vi "Repeat.vi"(11 "CSM Name":string="Repeat") -> ()   [LabVIEW 2026, in "UI-步进.lvlib" / "Repeat.lvlib"]
uses:
  Repeat.lvlib
  Supports/Repeat Steps.ctl
  Supports/Repeating States.ctl
  <userlib>/_NEVSTOP/Communicable State Machine(CSM)/_Polymophic/CSM - Filter Duplicated Lines.vi
  816fba94-53db-458f-9fde-c2796c7a1569.vi
  ea879a80-eb10-4c3f-a93b-bc01ba185342.vi
  ba2d9a0e-10df-4741-bda9-2194bb22ae09.vi
  84c4a0cb-90b1-43d3-96e0-8d2f37924e74.vi
  ccb58757-6b9e-4b1a-98c8-8aa3e3073145.vi
  b9097fe4-5901-4bf7-874c-569f3441d03a.vi
  be3ae19b-8a37-463e-a95d-eee2ed27764c.vi
  05157bae-8af7-4530-8df5-f99514427171.vi
  <userlib>/_NEVSTOP/Communicable State Machine(CSM)/_Polymophic/CSM - Replace Marks in Messages.vi
  2c826c22-9728-4daa-abad-67d06329c265.vi
  1395e5c4-d7de-483e-aee6-084de6ff1113.vi
  <userlib>/_NEVSTOP/Communicable State Machine(CSM)/AdvanceAPI/CSM - Compact Multiple States.vi
  <userlib>/_NEVSTOP/Communicable State Machine(CSM)/AdvanceAPI/CSM - Break Down Multiple States String.vi
  <userlib>/_NEVSTOP/Communicable State Machine(CSM)/_Shared/Remove Comments from Single-line.vi
  <userlib>/_NEVSTOP/Communicable State Machine(CSM)/_Shared/Split Single-line Message.vi
  <userlib>/_NEVSTOP/Communicable State Machine(CSM)/_Shared/Trim Single-line Text.vi
  <userlib>/_NEVSTOP/Communicable State Machine(CSM)/AdvanceAPI/CSM - Revert Arguments-Safe String.vi
  <userlib>/_NEVSTOP/Communicable State Machine(CSM)/AdvanceAPI/CSM - Make String Arguments Safe.vi
  <userlib>/_NEVSTOP/Communicable State Machine(CSM)/AdvanceAPI/CSM - Keywords.vi
  <userlib>/_NEVSTOP/Communicable State Machine(CSM)/AdvanceAPI/CSM - Get Module Attribute.vi
  <userlib>/_NEVSTOP/Communicable State Machine(CSM)/addons/API-String-Arugments-Support/_Support/Convert API String Arguments to Data(variant).vi
  <userlib>/_NEVSTOP/Communicable State Machine(CSM)/addons/API-String-Arugments-Support/_Support/Data To API String Arguments.vi
  <userlib>/_NEVSTOP/Communicable State Machine(CSM)/Communicable State Machine.lvlib
  <userlib>/_NEVSTOP/Communicable State Machine(CSM)/addons/Loop-Support/CSM Loop Support.lvlib
  <userlib>/_NEVSTOP/Communicable State Machine(CSM)/addons/INI-Static-Variable-Support/INI-Static-Variable-Support.lvlib
panel:
  in  "运行次数":dbl=inf format="%#.0f"
  out "当前次数":i32
  in  "循环开始":bool
  in  "电机步骤":T1=[{"行程"=25, "周期"=600, "进度"=0.0, "光谱测量拿起"=FALSE, "运行方向"=FALSE}, {"行程"=25, "周期"=600, "进度"=0.0, "光谱测量拿起"=FALSE, "运行方向"=FALSE}, {"行程"=25, "周期"=600, "进度"=0.0, "光谱测量拿起"=FALSE, "运行方向"=FALSE}, {"行程"=25, "周期"=600, "进度"=0.0, "光谱测量拿起"=FALSE, "运行方向"=FALSE}] {"进度" scale=0.0..1.0}
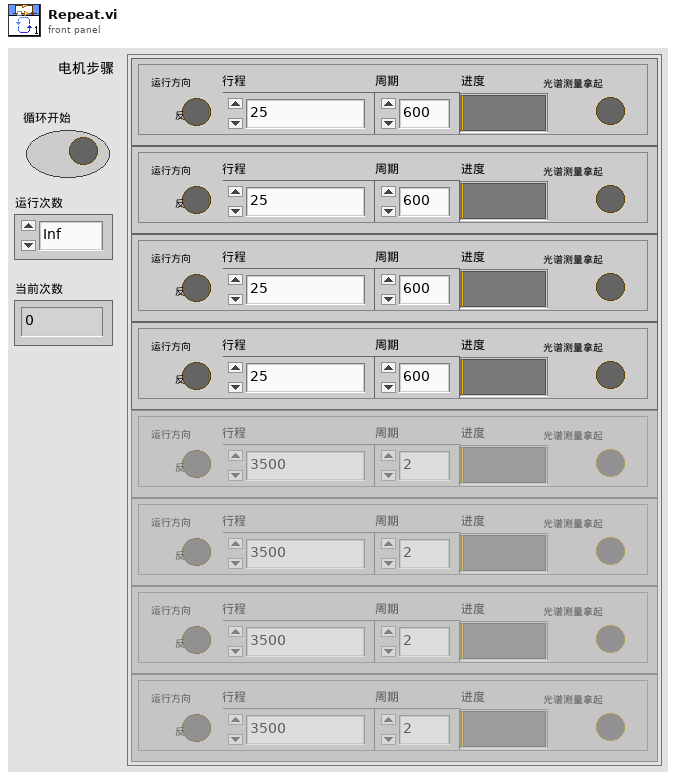
[diagram p1: front panel]
types:
  T1 = typedef "UI-步进.lvlib/Repeat Steps.ctl" = cluster{"行程":i32, "周期":i32, "进度":dbl, "光谱测量拿起":bool, "运行方向":bool}[]
  T2 = enum32{"Invalid", "Standard", "Closed", "Hidden", "Minimized", "Maximized"}
  T3 = enum32{"invalid app kind", "Development System", "Run Time System", "Student Edition", "Embedded LabVIEW", "Evaluation", "Custom"}
  T4 = typedef "UI-步进.lvlib/Repeat.lvlib/Repeating States.ctl" = enum16{"Idle", "Repeating", "Error"}
  T5 = typedef "Communicable State Machine.lvlib/_CSM_Response Source Message.ctl" = cluster{"‘State":string, "’Arguments":string, "’Error":errorcluster}
  T6 = cluster{"Current VI Reference":refnum<vi>, "Close Panel on Exit?":bool}
  T7 = cluster{"Core":cluster{"Current VI Reference":refnum<vi>, "Close Panel on Exit?":bool}, "State":T4, "Repeat":cluster{"电机步骤开始时间":timestamp, "电机步骤索引":i32[], "下一步？":bool, "步骤开始周期":i32}, "CSM Name":string, "INI Path":path}
  T8 = cluster{"电机步骤开始时间":timestamp, "电机步骤索引":i32[], "下一步？":bool, "步骤开始周期":i32}
  T9 = cluster{"行程":i32, "周期":i32, "进度":dbl, "光谱测量拿起":bool, "运行方向":bool}
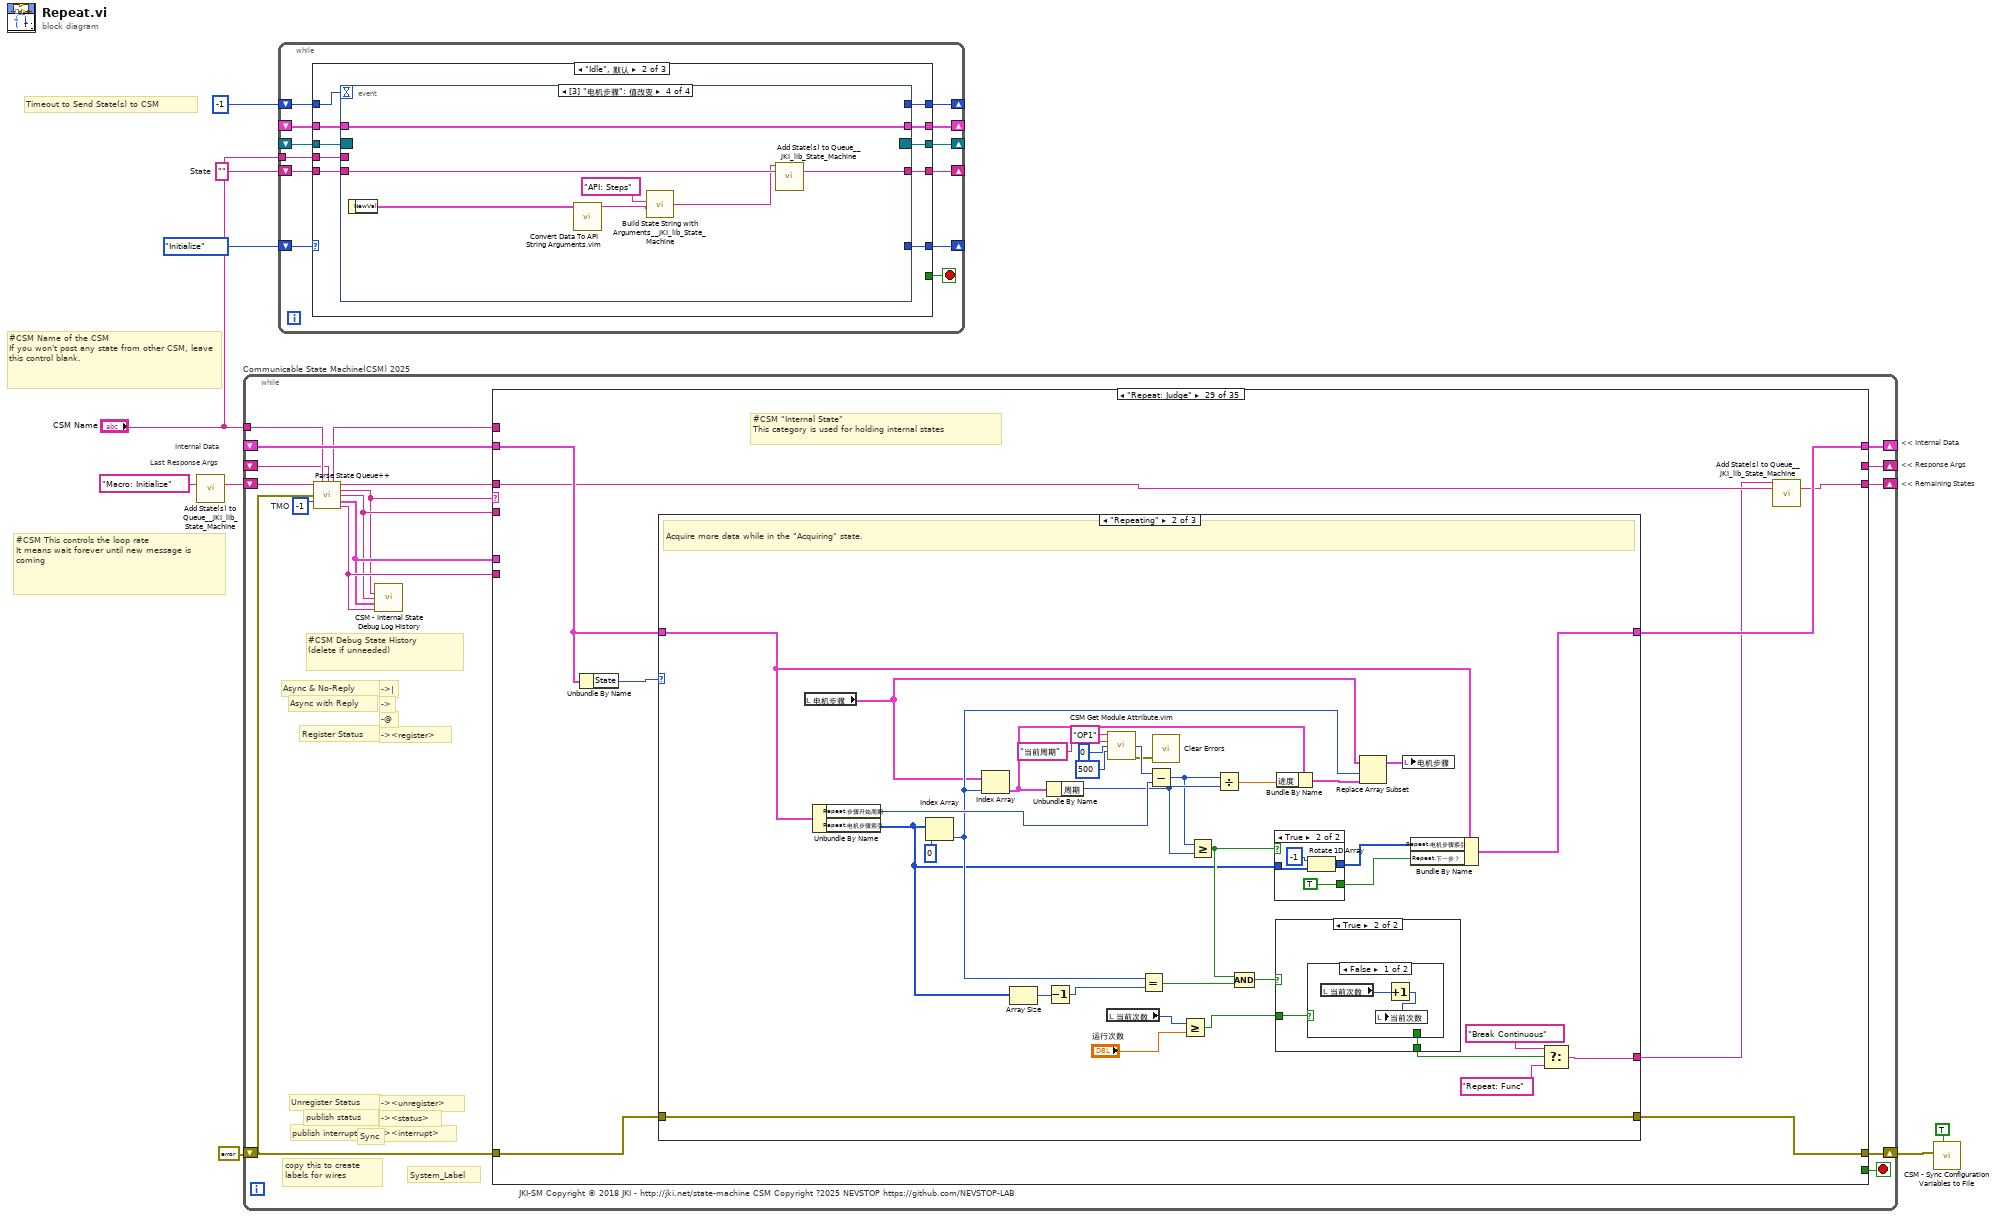
[diagram p0: block diagram]
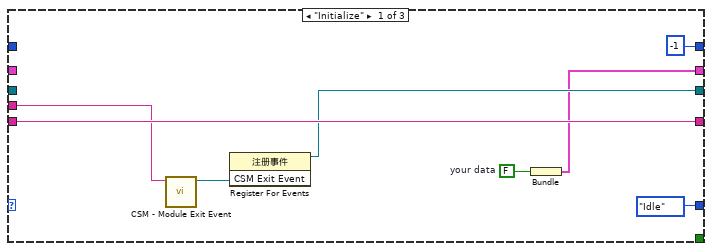
[diagram p2: hidden frame]
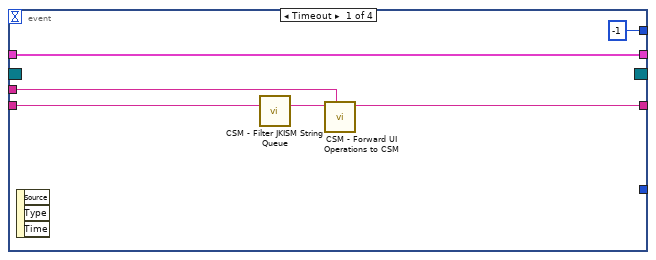
[diagram p3: hidden frame]
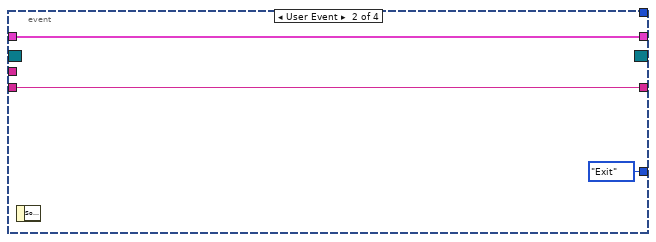
[diagram p4: hidden frame]
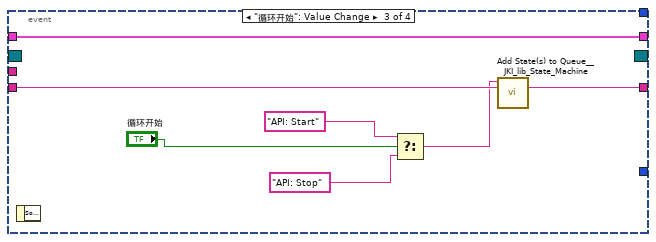
[diagram p5: hidden frame]
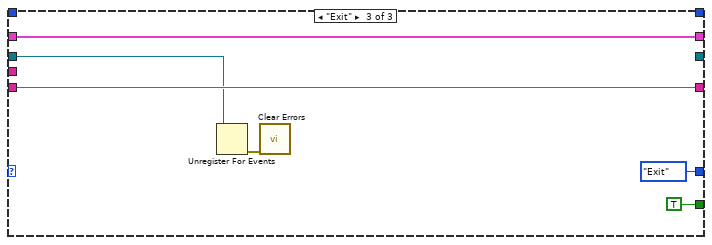
[diagram p6: hidden frame]
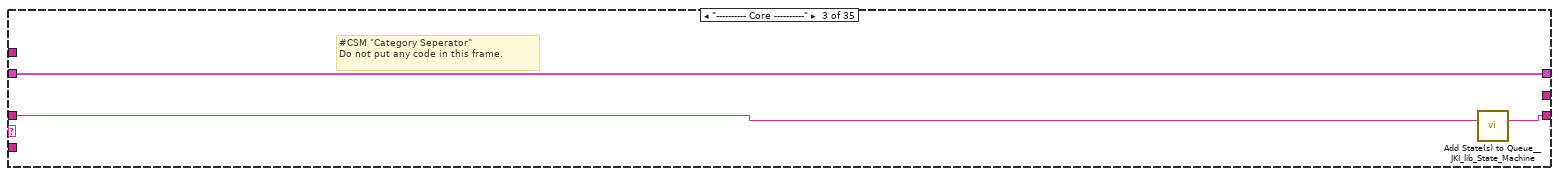
[diagram p9: hidden frame]
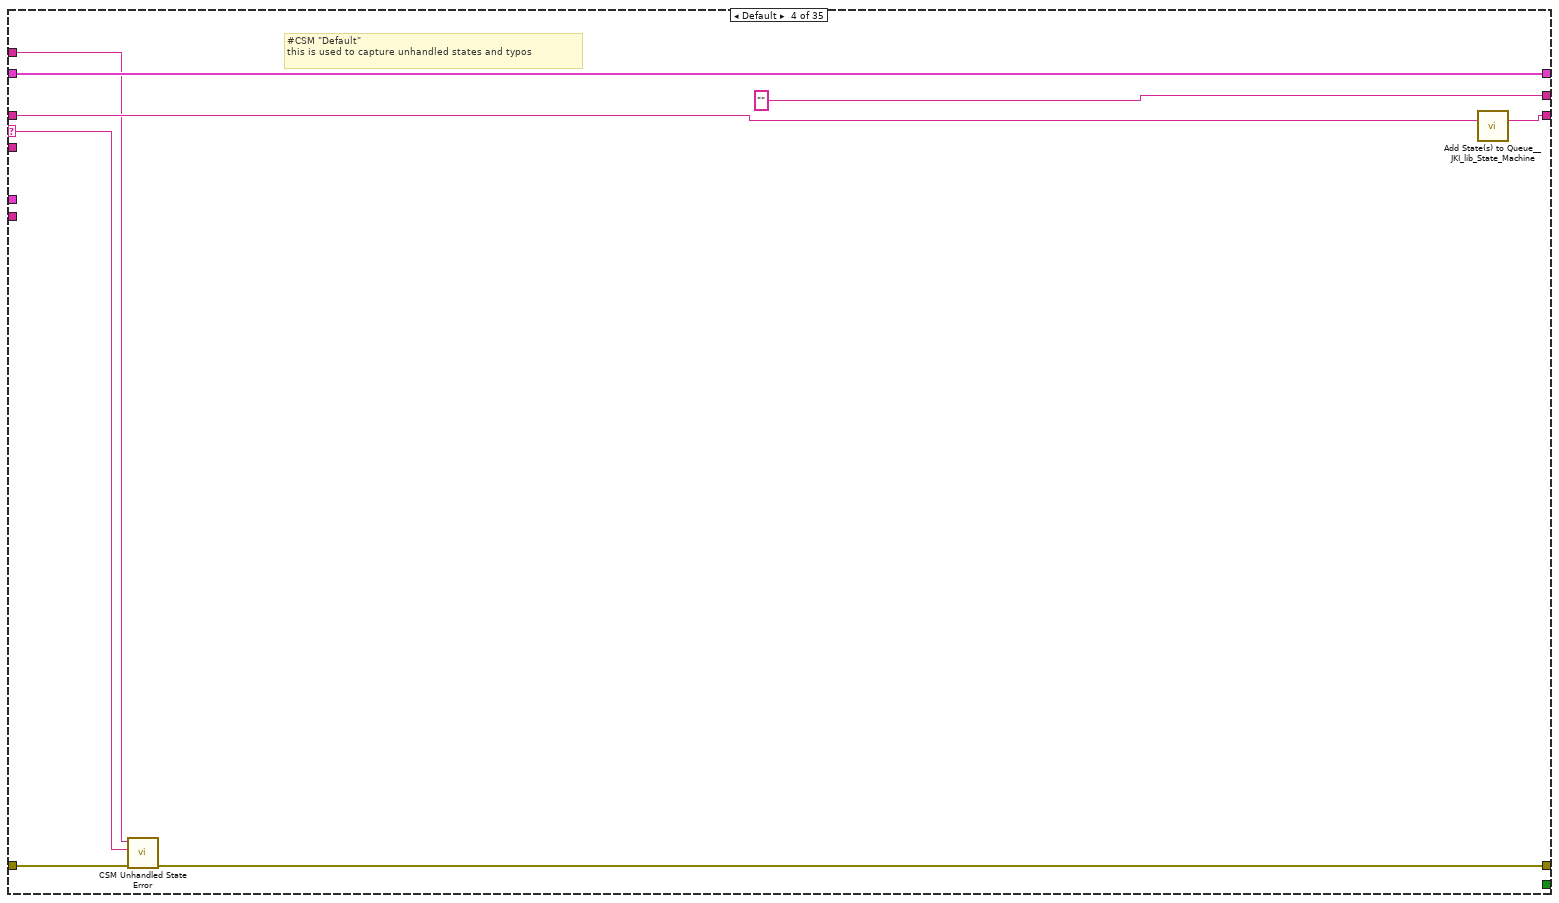
[diagram p10: hidden frame]
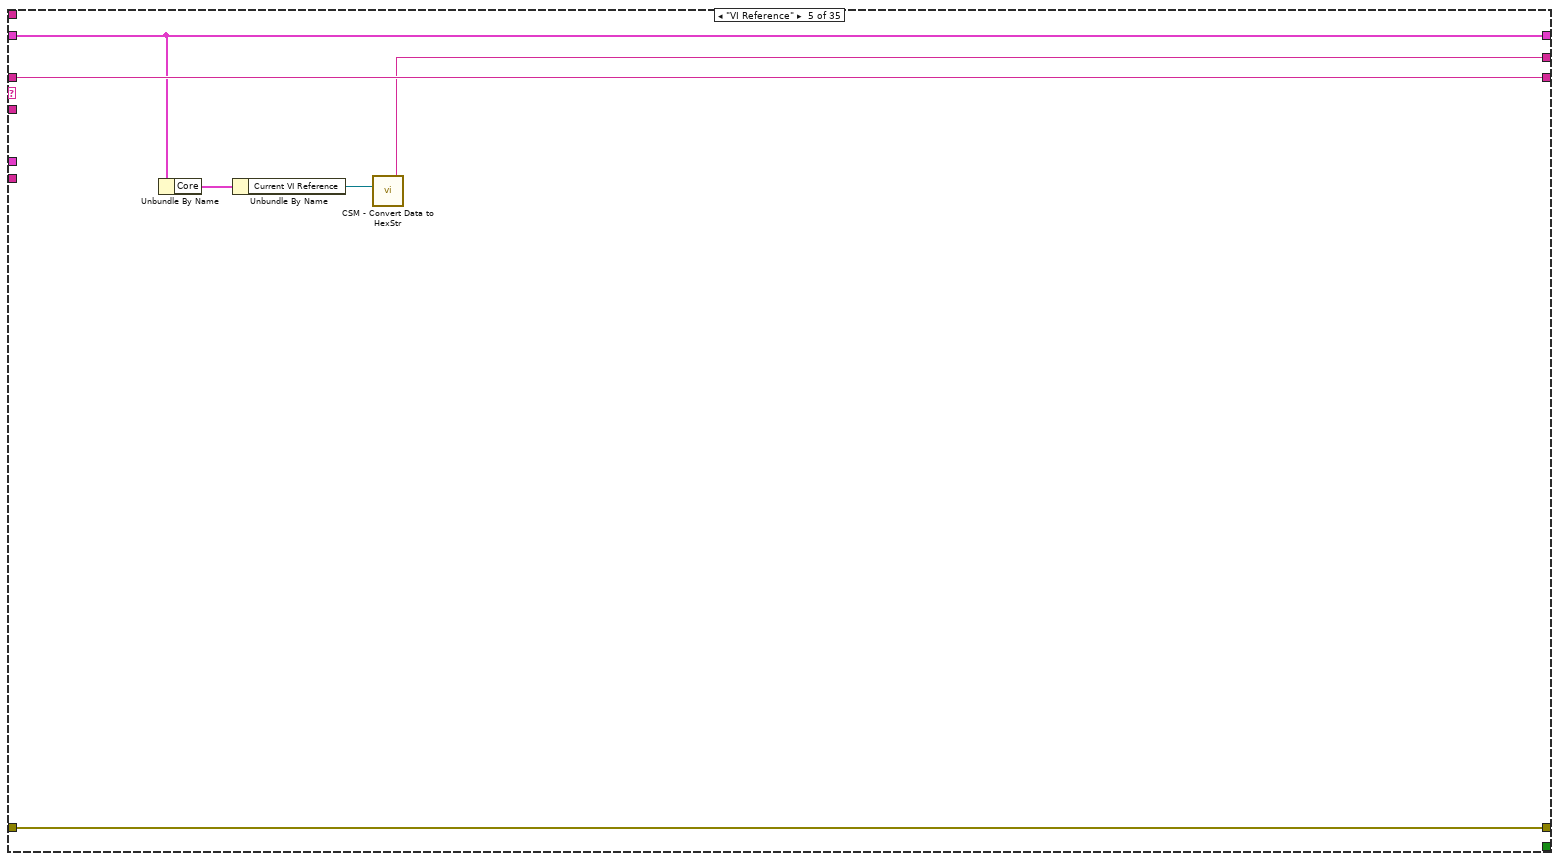
[diagram p11: hidden frame]
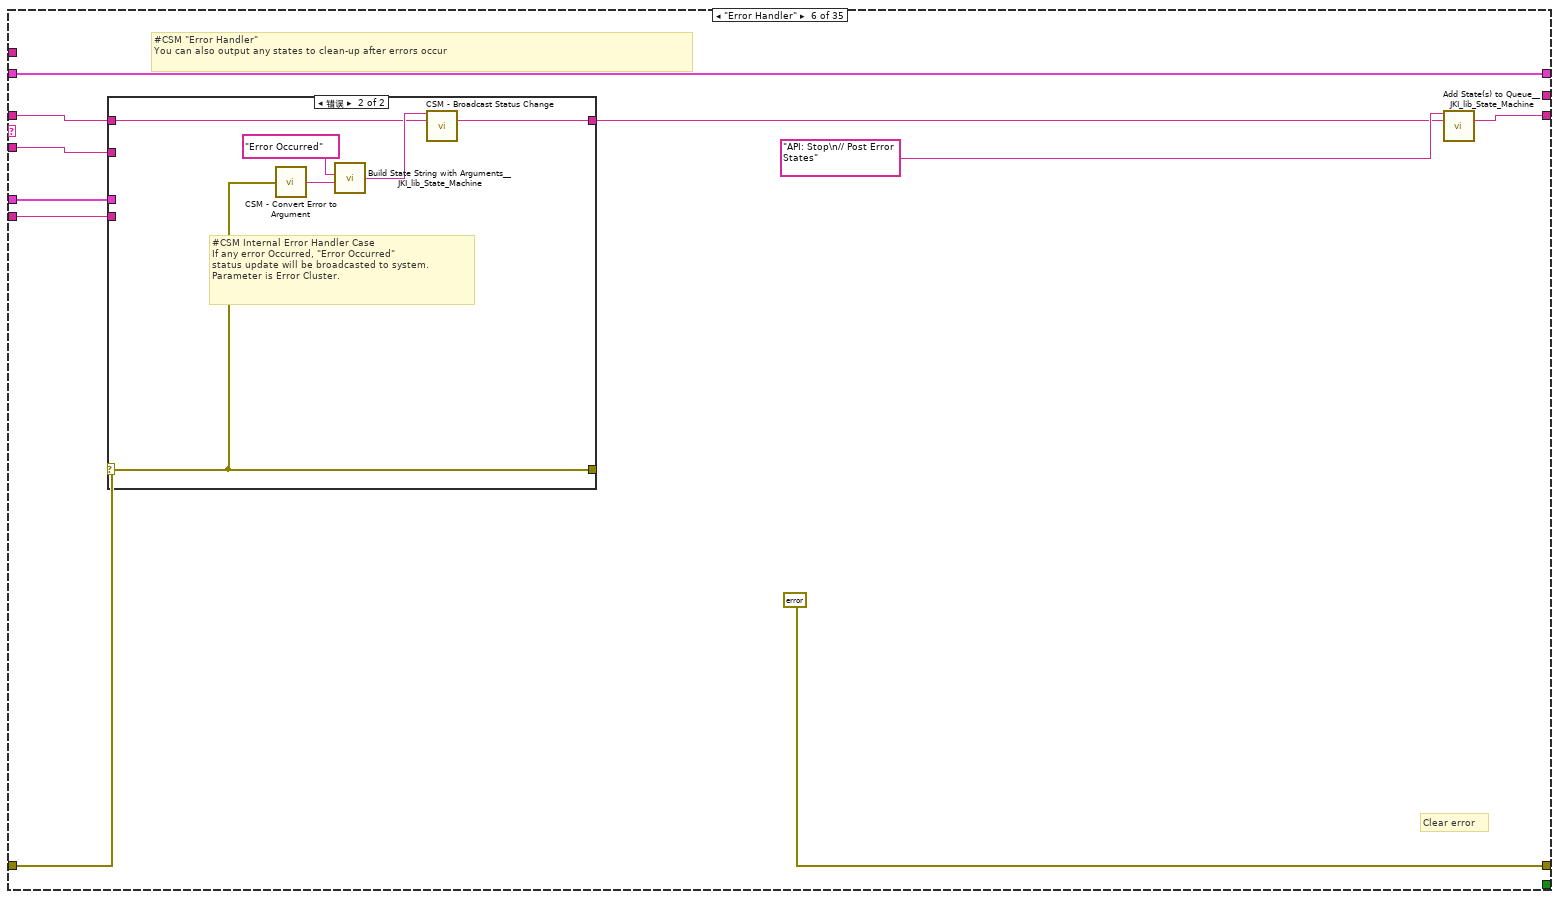
[diagram p12: hidden frame]
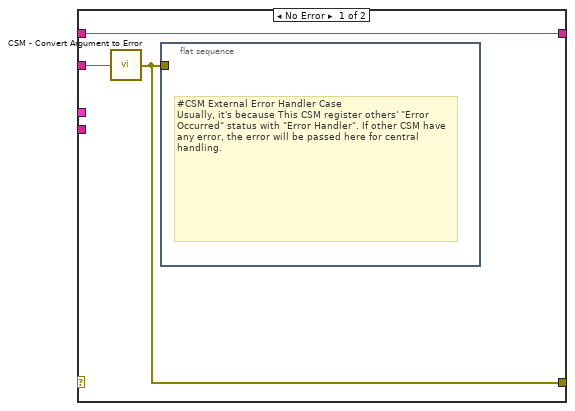
[diagram p13: hidden frame]
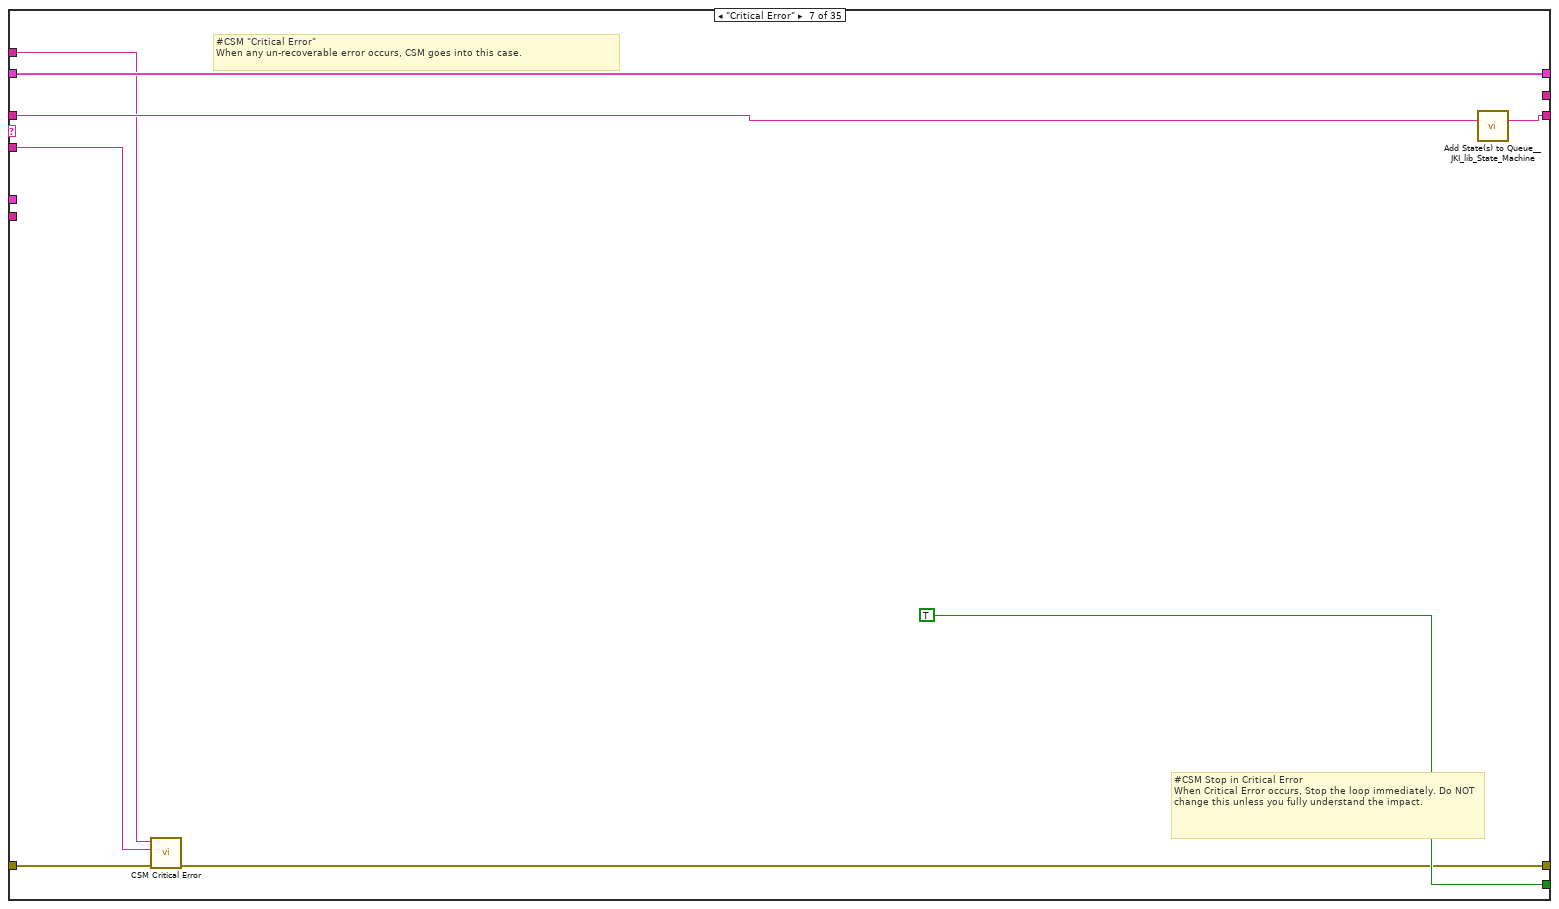
[diagram p14: hidden frame]
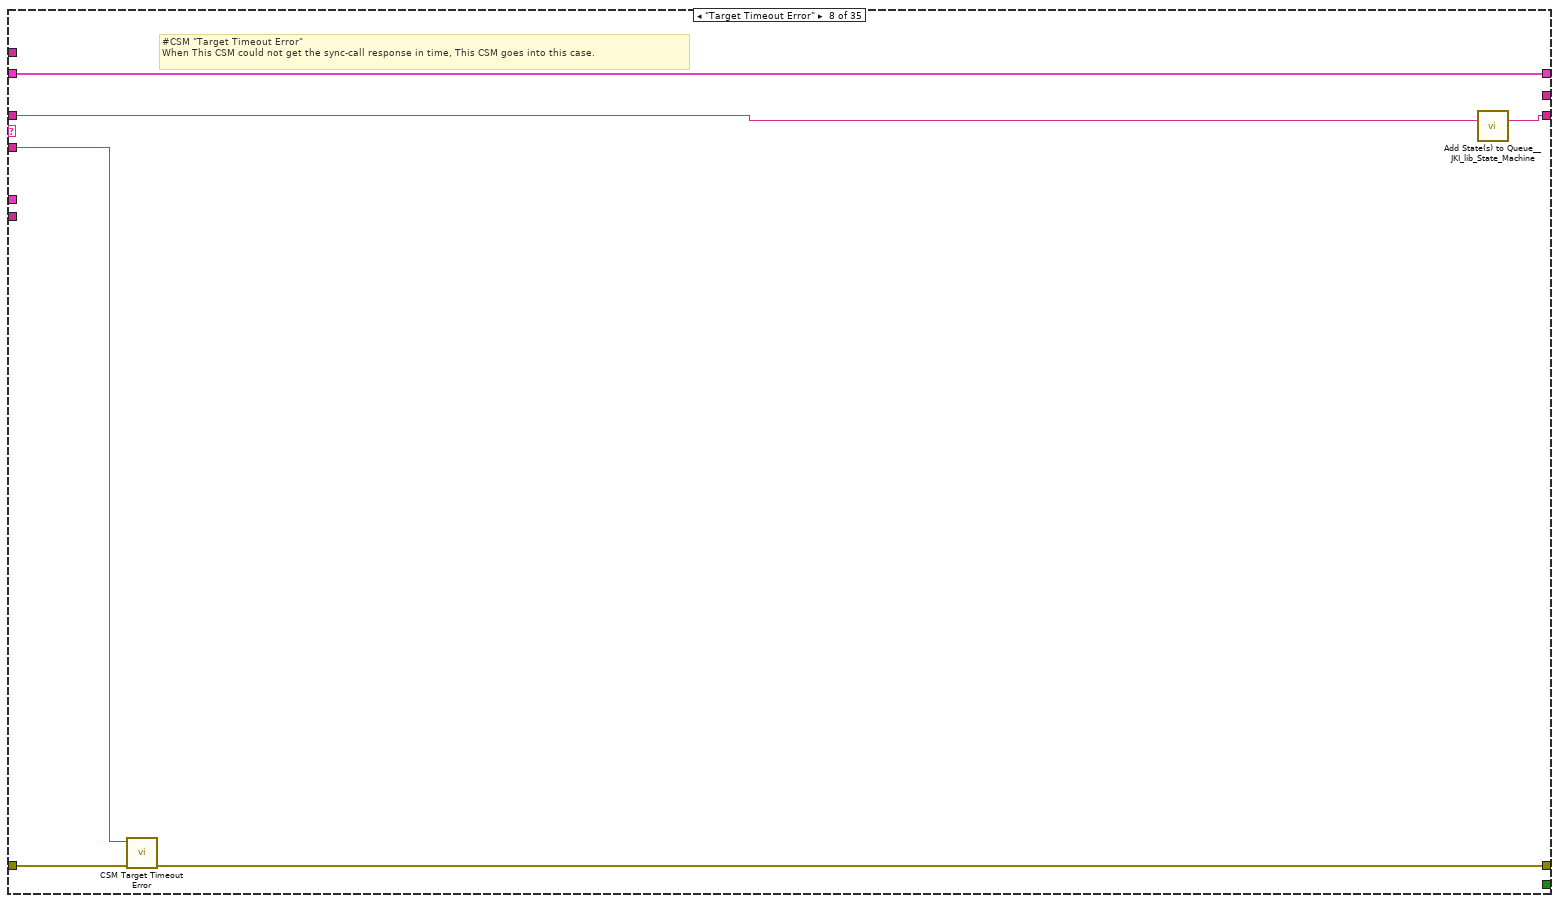
[diagram p15: hidden frame]
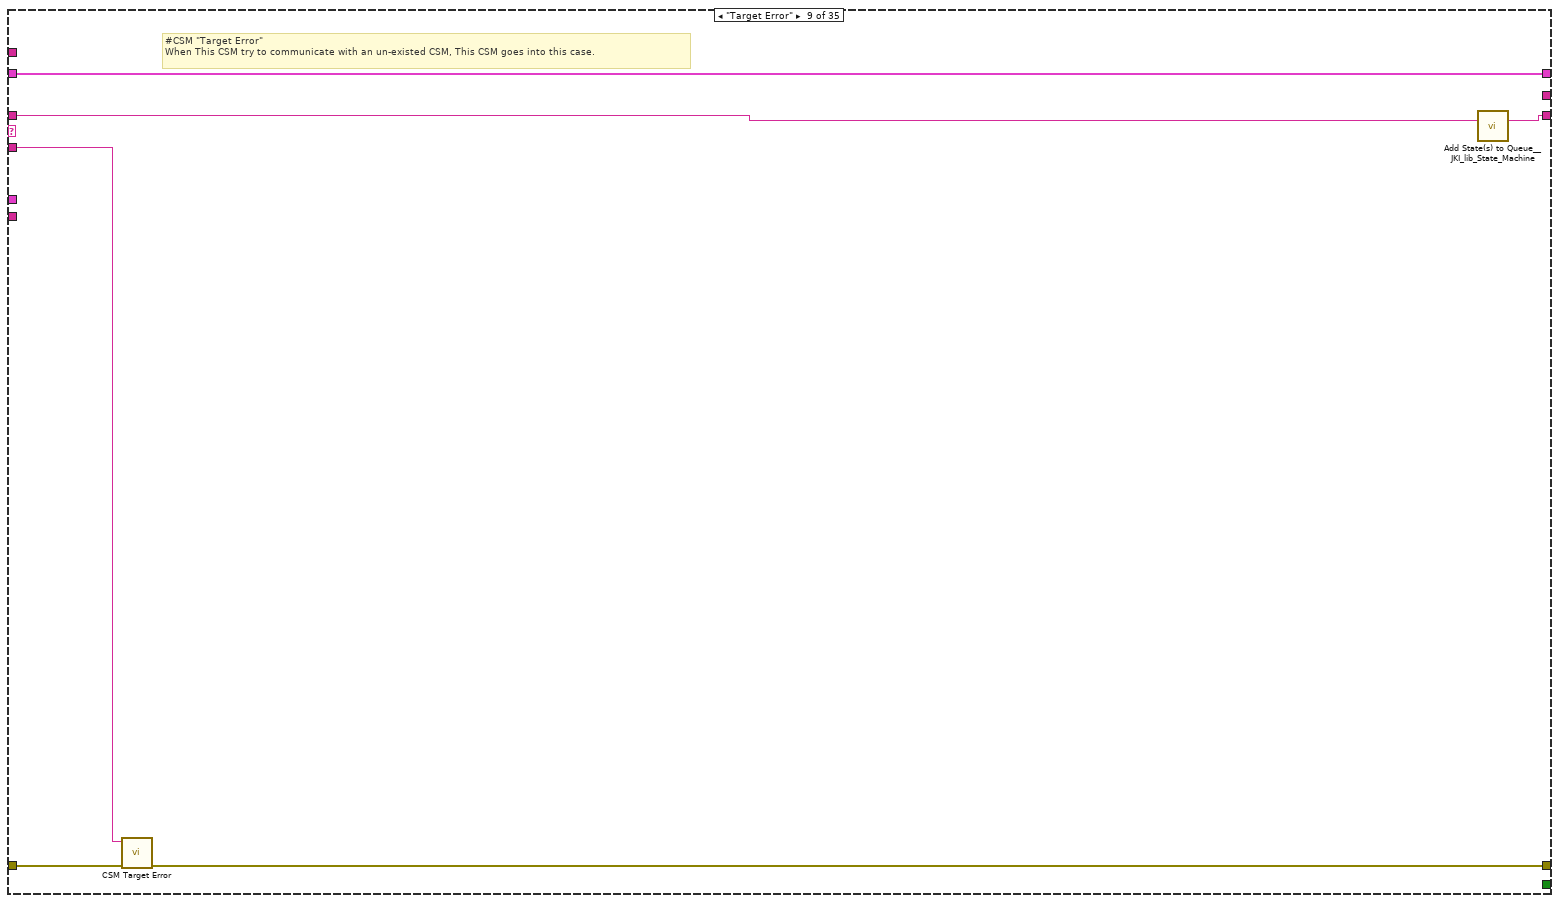
[diagram p16: hidden frame]
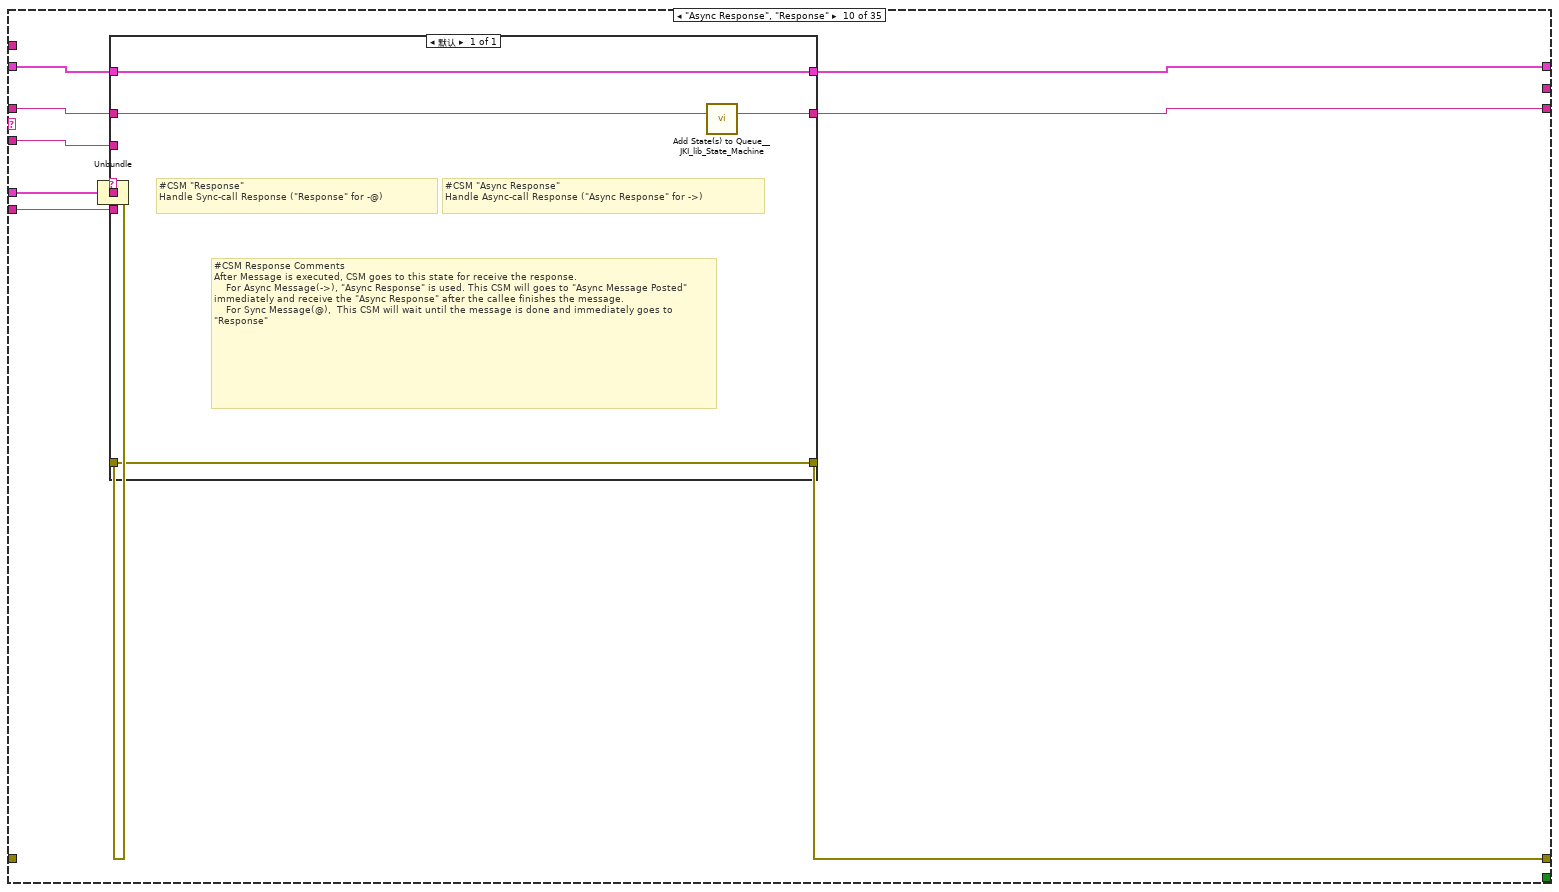
[diagram p17: hidden frame]
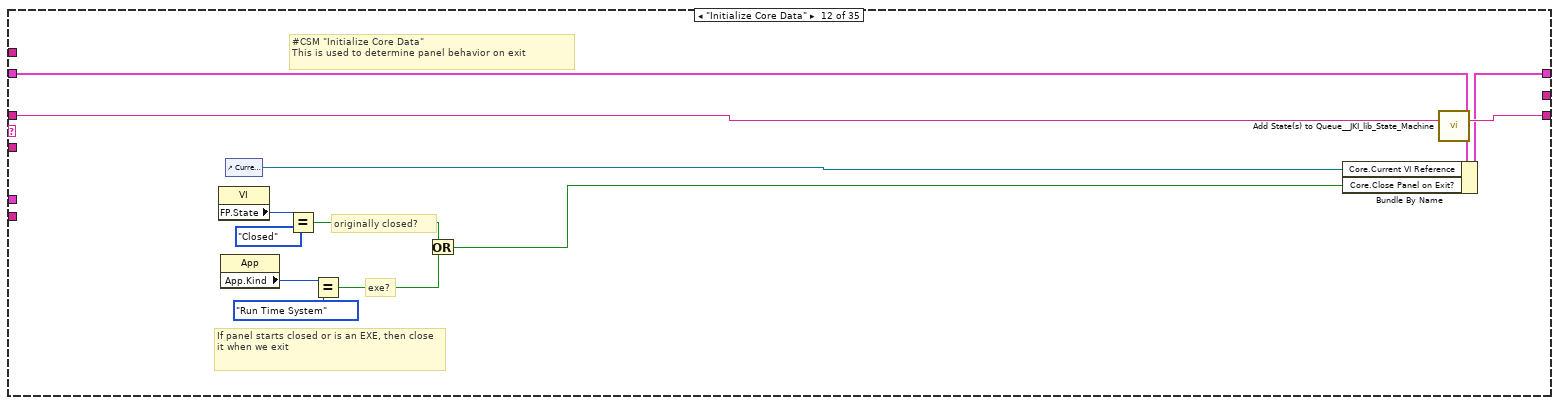
[diagram p19: hidden frame]
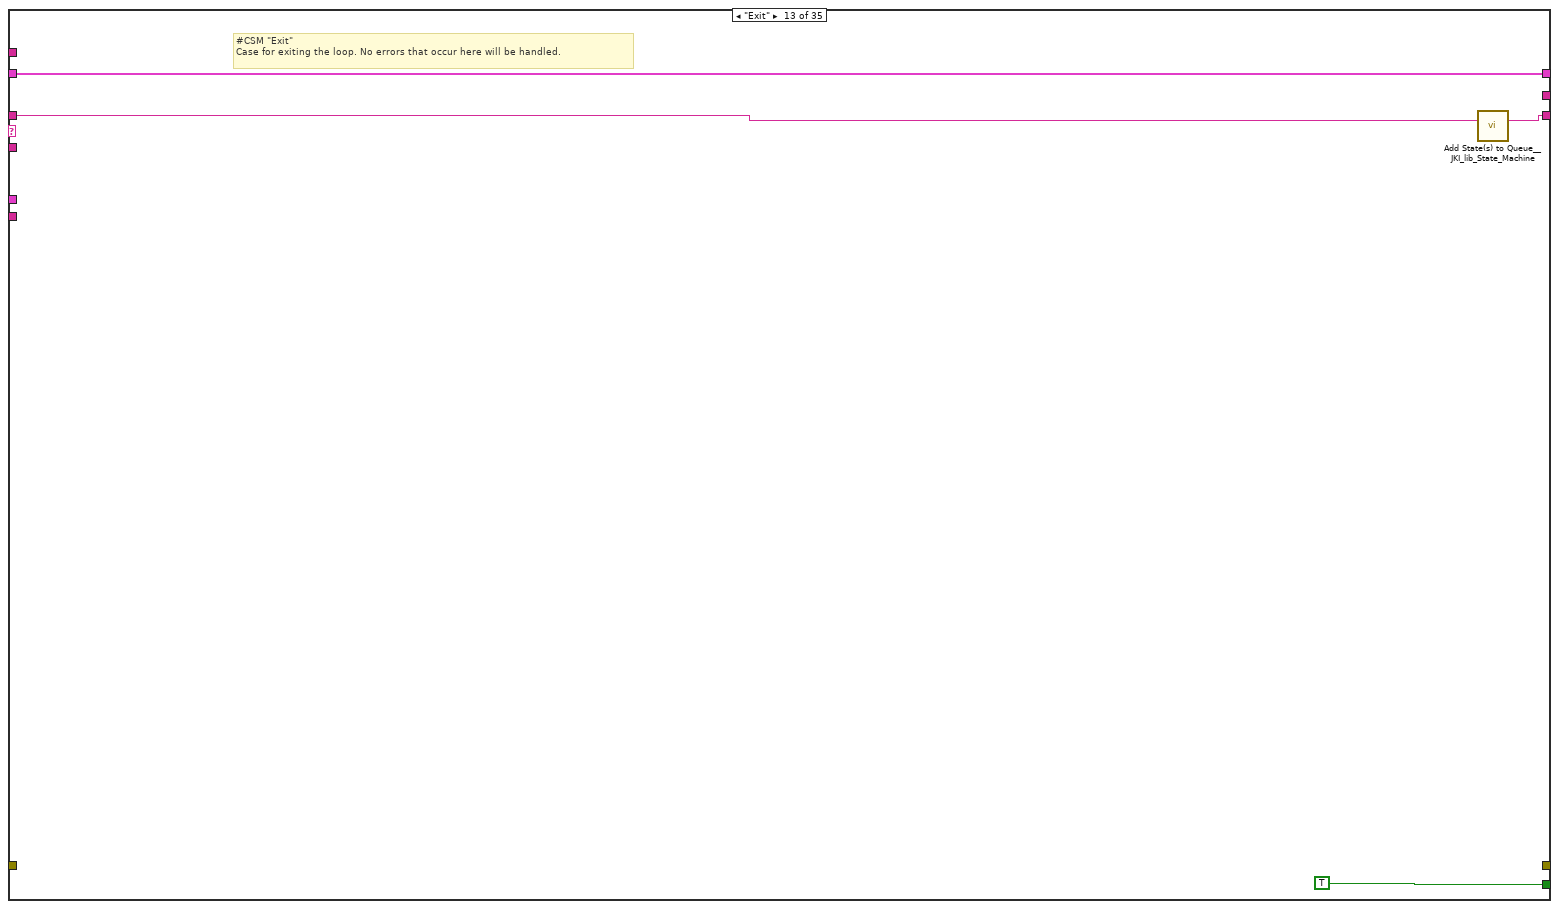
[diagram p20: hidden frame]
diagram:
  w5 = ""  # State
  # "Timeout to Send State(s) to CSM"
  # "Last Response Args"
  # "Internal Data"
  # "#CSM Name of the CSM\nIf you won't post any state from other CSM, leave this control blank."
  # "#CSM This controls the loop rate\nIt means wait forever until new message is coming"
  # "<< Internal Data"
  # "<< Response Args"
  # "<< Remaining States"
  n1 = call <vilib>:"Add State(s) to Queue__JKI_lib_State_Machine.vi"("State(s) in (\"\")"="Macro: Initialize" ("Init State(\"Macro: Initialize\")")) -> ("States Out"=w7:string)  [unwired: 14 in]
  n2 = while "Communicable State Machine(CSM) 2025" {
    shift-right: [w21] -> _
    shift-left: _ -> [w20]
    shift-right: [w24] -> w2
    shift-left: errorcluster {"status"=FALSE, "code"=0, "source"=""} ("error out") -> [w10]
    shift-right: [w23] -> _
    shift-left: w7 -> [w25]
    tunnel: "CSM Name" -> [w17]
    shift-right: [w18] -> _
    shift-left: _ -> [w12]
    stop <- w22 stop-if-true
    w19 = -1  # TMO
    # "#CSM Debug State History\n(delete if unneeded)"
    # "-><interrupt>"
    # "-><status>"
    # "-><unregister>"
    # "-><register>"
    # "-@"
    # "->"
    # "->|"
    # "publish interrupt"
    # "publish status"
    # "Unregister Status"
    # "Register Status"
    # "Sync"
    # "Async with Reply"
    # "Async & No-Reply"
    # "JKI-SM Copyright © 2018 JKI - http://jki.net/state-machine CSM Copyright ?2025 NEVSTOP https://github.com/NEVSTOP-LAB"
    # "copy this to create labels for wires"
    # "System_Label"
    n3 = call <userlib>:"Parse State Queue++.vi"("State Queue"=w25, "Name (\"\" to Use UUID)"=w17, "Response Arguments"=w12, "Previous Error"=w10, "Dequeue (1 ms)"=w19) -> ("Name Used"=w11:string, "Remaining States"=w26:string, "Current State"=w13:string, "Arguments"=w14:string, "Additional Information"=w15:T5, "Source CSM"=w16:string)  [unwired: 5 in]
    n4 = call <userlib>:"CSM - Internal State Debug Log History.vi"("State"=w13, "Arguments (\"\")"=w14, ">> Response Source Message >>"=w15, "Source (\"\")"=w16) -> ()  [unwired: 11 in, 1 out]
    n5 = case shown="\"Repeat: Judge\"" w13 {
      selector: w13 -> [_ _ _ w37 _ _ _ _ _ _ _ _ _ _ _ _ _ _ _ _ _ _ _ _ _ _ _ _ _ _ _ _ _ w393 _]
      tunnel: w26 -> [w27 w30 w33 w41 w46 w51 w74 w80 w86 w96 w103 w115 w119 w122 w130 w133 w139 w142 w146 w154 w159 w165 w187 w194 w198 w207 w211 w216 w241 w303 w381 w386 w389 w394 w398]
      tunnel: w14 -> [_ _ _ _ _ w50 w70 w77 w83 w90 _ _ _ _ _ _ _ _ _ _ _ _ _ w193 w196 w206 _ _ _ _ _ _ _ w391 _]
      tunnel: w20 -> [w28 w29 w31 w39 w45 w56 w72 w78 w84 w94 w102 w109 w117 w120 _ w132 w135 w140 w144 w147 w160 w163 w188 w192 w201 w204 w209 w220 w246 w307 w379 w384 w387 w395 w397]
      tunnel: [_ _ _ w34 w47 errorcluster {"status"=FALSE, "code"=0, "source"=""} ("error out") w67 w75 w81 w97 _ _ _ _ _ _ w136 _ _ _ _ _ _ w195 w202 w208 _ _ w243 w321 _ _ _ _ w399] -> w24
      tunnel: w10 -> [_ _ _ w35 w47 w54 w68 w76 w82 _ _ _ _ _ _ _ w134 _ _ _ _ _ _ w195 w202 w208 _ _ w245 w321 _ _ _ _ w399]
      tunnel: [w27 w30 w32 w40 w46 w52 w73 w79 w85 w95 w103 w114 w118 w121 w129 w133 w138 w141 w145 w153 w158 w164 w186 w194 w197 w207 w210 w217 w242 w304 w380 w385 w388 w392 w396] -> w23
      tunnel: [_ _ _ _ _ _ TRUE _ _ _ _ _ TRUE _ _ _ _ _ _ _ _ _ _ _ _ _ _ _ _ _ _ _ _ _ _] -> w22
      tunnel: [w28 w29 w31 w39 w45 w56 w72 w78 w84 w93 w102 w113 w117 w120 w128 w132 w135 w140 w144 w147 w160 w166 w188 w191 w201 w204 w209 w227 w244 w306 w379 w383 w387 w395 w397] -> w21
      tunnel: w16 -> [_ _ _ _ _ w49 _ _ _ w91 _ _ _ _ _ _ _ _ _ _ _ _ _ _ _ _ _ _ _ _ _ _ _ _ _]
      tunnel: w15 -> [_ _ _ _ _ w48 _ _ _ w92 _ _ _ _ _ _ _ _ _ _ _ _ _ _ _ _ _ _ _ _ _ _ _ _ _]
      tunnel: [_ _ _ "" w42 _ _ _ _ _ _ _ _ _ _ _ _ _ _ _ _ _ _ _ _ _ _ _ _ _ _ _ _ _ _] -> w18
      tunnel: w11 -> [_ _ _ w36 _ _ w69 _ _ _ _ _ _ _ _ _ _ _ _ _ _ _ _ _ _ _ _ _ _ _ _ _ _ _ _]
      frame "", "Idle" {
        # "#CSM \"Idle/Event Handler\"\nexecutes when the state queue is empty"
      }
      frame "CSM Documentation" {
        # "#CSM State Syntax\n\n// Comment line, all text to the right of “//” will be ignored\n// Local Message Example\nDoSth: DoA >> Arguments\n\n// Sync Call Example\nAPI: xxxx >> Arguments -@ TargetModule\n\n// Async Call Example\nAPI: xxxx >> Arguments -> TargetModule\n\n// Async Call without Reply Example\nAPI: xxxx >> Arguments ->| TargetModule\n\n// Broadcast normal status:\nStatus >> StatusArguments  -><status>\n\n// Broadcast Interrupt status:\nInterrupt >> StatusArguments  -><interrupt>\n\n// Register Source Module's status to Handler Module\nStatus@Source Module >> Handler Module@Handler Module -><register>\n\n// Unegister Source Module's status\nStatus@Source Module >> Handler Module -><unregister>"
        # "#CSM README FIRST\n\nCommunicable State Machine(CSM) is a LabVIEW application framework that builds upon JKI State Machine(JKISM). It follows the pattern of JKISM and extends the keywords to describe message communication between modules, including concepts such as Sync-Message, Async-Message, Subscription/Unsubscription of status - essential elements for creating reusable code modules. For more information, please visit the CSM wiki: https://nevstop-lab.github.io/CSM-Wiki/\n\nFor instructions on JKI State Machine, visit: \n    http://jki.net/state-machine/\nFor information about CSM, visit: \n    https://github.com/NEVSTOP-LAB"
        # "#CSM \"Documentation\"\nCase for holding CSM Documenation"
      }
      frame "---------- Core ----------" {
        # "#CSM \"Category Seperator\"\nDo not put any code in this frame."
        n6 = call <vilib>:"Add State(s) to Queue__JKI_lib_State_Machine.vi"("State(s) in (\"\")"=w33) -> ("States Out"=w32:string)  [unwired: 14 in]
      }
      frame Default {
        # "#CSM \"Default\"\nthis is used to capture unhandled states and typos"
        n7 = call <userlib>:"CSM Unhandled State Error.vi"("error in (no error)"=w35, "Undefined State"=w37, "CSM Name"=w36) -> ("error out"=w34:errorcluster)  [unwired: 8 in]
        n8 = call <vilib>:"Add State(s) to Queue__JKI_lib_State_Machine.vi"("State(s) in (\"\")"=w41) -> ("States Out"=w40:string)  [unwired: 14 in]
      }
      frame "VI Reference" {
        n9 = Unbundle By Name(w45) -> ("Core"=w44:T6)
        n10 = Unbundle By Name(w44) -> ("Current VI Reference"=w43:refnum<vi>)
        n11 = call <userlib>:"CSM - Convert Data to HexStr.vi"("Variant"=w43) -> ("HEX String (0-9,A-F)"=w42:string)  [unwired: 8 in]
      }
      frame "Error Handler" {
        # "#CSM \"Error Handler\"\nYou can also output any states to clean-up after errors occur"
        # "Clear error"
        n12 = case shown="错误" w54 {
          selector: w54 -> [_ w61]
          tunnel: [w60 w63] -> w53
          tunnel: w51 -> [w60 w62]
          tunnel: w50 -> [w59 _]
          tunnel: w49 -> [_ _]
          tunnel: w48 -> [_ _]
          tunnel: [w58 w61] -> _
          frame No Error {
            n13 = call <userlib>:"CSM - Convert Argument to Error.vi"("Argument"=w59) -> ("Error"=w58:errorcluster)  [unwired: 4 in]
            n14 = flat-sequence {
              tunnel: w58 -> [_]
              frame #0 {
                # "#CSM External Error Handler Case\nUsually, it's because This CSM register others' \"Error Occurred\" status with \"Error Handler\". If other CSM have any error, the error will be passed here for central handling."
              }
            }
          }
          frame Error {
            # "#CSM Internal Error Handler Case \nIf any error Occurred, \"Error Occurred\" \nstatus update will be broadcasted to system.\nParameter is Error Cluster."
            n15 = call <userlib>:"CSM - Convert Error to Argument.vi"("Error"=w61) -> ("Argument"=w65:string)  [unwired: 4 in]
            n16 = call <vilib>:"Build State String with Arguments__JKI_lib_State_Machine.vi"("Arguments (\"\")"=w65, "State"="Error Occurred" ("Status with Arguments")) -> ("State with Arguments"=w64:string)  [unwired: 4 in]
            n17 = call <userlib>:"CSM - Broadcast Status Change.vi"("Status With Arguments"=w64, "State Queue"=w62) -> ("Remaining States"=w63:string)  [unwired: 13 in]
          }
        }
        n18 = call <vilib>:"Add State(s) to Queue__JKI_lib_State_Machine.vi"("State(s) in Front (\"\")"="API: Stop\n// Post Error States", "State(s) in (\"\")"=w53) -> ("States Out"=w52:string)  [unwired: 13 in]
      }
      frame "Critical Error" {
        # "#CSM \"Critical Error\"\nWhen any un-recoverable error occurs, CSM goes into this case."
        # "#CSM Stop in Critical Error\nWhen Critical Error occurs, Stop the loop immediately. Do NOT change this unless you fully understand the impact."
        n19 = call <userlib>:"CSM Critical Error.vi"("error in (no error)"=w68, "Arugments (As Reason)"=w70, "CSM Name"=w69) -> ("error out"=w67:errorcluster)  [unwired: 8 in]
        n20 = call <vilib>:"Add State(s) to Queue__JKI_lib_State_Machine.vi"("State(s) in (\"\")"=w74) -> ("States Out"=w73:string)  [unwired: 14 in]
      }
      frame "Target Timeout Error" {
        # "#CSM \"Target Timeout Error\"\nWhen This CSM could not get the sync-call response in time, This CSM goes into this case."
        n21 = call <userlib>:"CSM Target Timeout Error.vi"("error in (no error)"=w76, "Arguments (As CSM Name)"=w77) -> ("error out"=w75:errorcluster)  [unwired: 9 in]
        n22 = call <vilib>:"Add State(s) to Queue__JKI_lib_State_Machine.vi"("State(s) in (\"\")"=w80) -> ("States Out"=w79:string)  [unwired: 14 in]
      }
      frame "Target Error" {
        # "#CSM \"Target Error\"\nWhen This CSM try to communicate with an un-existed CSM, This CSM goes into this case."
        n23 = call <userlib>:"CSM Target Error.vi"("error in (no error)"=w82, "Arguments (As CSM Name)"=w83) -> ("error out"=w81:errorcluster)  [unwired: 9 in]
        n24 = call <vilib>:"Add State(s) to Queue__JKI_lib_State_Machine.vi"("State(s) in (\"\")"=w86) -> ("States Out"=w85:string)  [unwired: 14 in]
      }
      frame "Async Response", "Response" {
        n25 = Unbundle(w92) -> ("‘State"=w89:string, "’Arguments"=w88:string, "’Error"=w87:errorcluster)
        n26 = case shown="默认" w89 {
          tunnel: [w98] -> w95
          tunnel: w96 -> [w99]
          tunnel: [w101] -> w93
          tunnel: w94 -> [w101]
          tunnel: [w100] -> w97
          tunnel: w87 -> [w100]
          tunnel: w91 -> [_]
          tunnel: w90 -> [_]
          tunnel: w88 -> [_]
          frame 默认 {
            # "#CSM \"Async Response\"\nHandle Async-call Response (\"Async Response\" for ->)"
            # "#CSM \"Response\"\nHandle Sync-call Response (\"Response\" for -@)"
            # "#CSM Response Comments\nAfter Message is executed, CSM goes to this state for receive the response.\n    For Async Message(->), \"Async Response\" is used. This CSM will goes to \"Async Message Posted\" immediately and receive the \"Async Response\" after the callee finishes the message.\n    For Sync Message(@),  This CSM will wait until the message is done and immediately goes to \"Response\""
            n27 = call <vilib>:"Add State(s) to Queue__JKI_lib_State_Machine.vi"("State(s) in (\"\")"=w99) -> ("States Out"=w98:string)  [unwired: 14 in]
          }
        }
      }
      frame "Async Message Posted" {
        # "#CSM \"Async Message Posted\"\nAfter Async Message is posted (-> or ->| ), CSM goes to this state for post-action.\nYou can use Argument - State to tell which Async Message is called."
      }
      frame "Initialize Core Data" {
        # "#CSM \"Initialize Core Data\"\nThis is used to determine panel behavior on exit"
        # "originally closed?"
        # "exe?"
        # "If panel starts closed or is an EXE, then close it when we exit"
        n28 = property class="VI"() -> ("FP.State"=w106:T2)  [unwired: 2 in, 2 out]
        n29 = property class="App"() -> ("App.Kind"=w112:T3)  [unwired: 2 in, 2 out]
        n30 = control-ref of="Current VI Reference"() -> (w107:refnum<vi>)
        n31 = Equal?(x=w106, y=T2."Closed" ("Front Panel Window:State")) -> (x = y?=w104:bool)
        n32 = Equal?(x=w112, y=T3."Run Time System" ("Application:Kind")) -> (x = y?=w110:bool)
        n33 = Or(x=w104, y=w110) -> (x .or. y?=w108:bool)
        n34 = Bundle By Name(cluster=w109, "Core.Current VI Reference"=w107, "Core.Close Panel on Exit?"=w108) -> (w113:T7)
        n35 = call <vilib>:"Add State(s) to Queue__JKI_lib_State_Machine.vi"("State(s) in (\"\")"=w115) -> ("States Out"=w114:string)  [unwired: 14 in]
      }
      frame "Exit" {
        # "#CSM \"Exit\"\nCase for exiting the loop. No errors that occur here will be handled."
        n36 = call <vilib>:"Add State(s) to Queue__JKI_lib_State_Machine.vi"("State(s) in (\"\")"=w119) -> ("States Out"=w118:string)  [unwired: 14 in]
      }
      frame "---------- Data ----------" {
        # "#CSM \"Category Seperator\"\nDo not put any code in this frame."
        n37 = call <vilib>:"Add State(s) to Queue__JKI_lib_State_Machine.vi"("State(s) in (\"\")"=w122) -> ("States Out"=w121:string)  [unwired: 14 in]
      }
      frame "Data: Initialize" {
        w123 = path ""  # INI Path
        w125 = ""  # CSM Name
        w124 = T8 {"电机步骤开始时间"=timestamp(0 s since 1904-01-01), "电机步骤索引"=[0, 1, 2, 3], "下一步？"=FALSE, "步骤开始周期"=0}  # Repeat
        w126 = Repeating_States."Idle"  # State
        w127 = T6 {"Current VI Reference"=refnum, "Close Panel on Exit?"=FALSE}  # Core
        # "#CSM \"Data: Initialize\"\nInitialize the shift-register data, here.\n(data names are defined by what you wire into the bundle function)"
        # "#CSM do not delete - used by framework"
        # "#CSM Data names and types of shift register data are defined by this bundle."
        n38 = Bundle("Core"=w127, "State"=w126, "Repeat"=w124, "CSM Name"=w125, "INI Path"=w123) -> (w128:T7)  [unwired: 1 in]
        n39 = call <vilib>:"Add State(s) to Queue__JKI_lib_State_Machine.vi"("State(s) in (\"\")"=w130) -> ("States Out"=w129:string)  [unwired: 14 in]
      }
      frame "Data: Update Indicators" {
        n40 = local write "循环开始"(FALSE ("循环开始")) -> ()
      }
      frame "Data: Cleanup" {
        # "#CSM \"Data: Cleanup\"\nCleanup any data and references, here.\n(this is called automatically, by the Macro: Exit)"
        n41 = Unbundle By Name(w135) -> ("Core.Current VI Reference"=w137:refnum<vi>)
        n42 = Close Reference(reference=w137, error in (no error)=w134) -> (error out=w136:errorcluster)
        n43 = call <vilib>:"Add State(s) to Queue__JKI_lib_State_Machine.vi"("State(s) in (\"\")"=w139) -> ("States Out"=w138:string)  [unwired: 14 in]
      }
      frame "---------- Macro ----------" {
        # "#CSM \"Category Seperator\"\nDo not put any code in this frame."
        n44 = call <vilib>:"Add State(s) to Queue__JKI_lib_State_Machine.vi"("State(s) in (\"\")"=w142) -> ("States Out"=w141:string)  [unwired: 14 in]
      }
      frame "Macro: Initialize" {
        # "#CSM \"Macro: Initialize\"\nInitialization Macro (This is called once, when the VI starts)"
        n45 = call <vilib>:"Add State(s) to Queue__JKI_lib_State_Machine.vi"("State(s) in Front (\"\")"="Data: Initialize\nInitialize Core Data\nData: Update Indicators", "State(s) in (\"\")"=w146) -> ("States Out"=w145:string)  [unwired: 13 in]
      }
      frame "Macro: Exit" {
        # "#CSM \"Macro: Exit\"\nExit Macro (This is called once, when the VI exits)"
        n46 = Unbundle By Name(w147) -> ("State"=w151:T4)
        n47 = case shown="\"Repeating\"" w151 {
          tunnel: ["" "Break Continuous\nRepeat: Close" ""] -> w149
          frame "Idle", Default {
          }
          frame "Repeating" {
          }
          frame "Error" {
          }
        }
        n48 = call <vilib>:"Add State(s) to Queue__JKI_lib_State_Machine.vi"("State(s) in Front (\"\")"="//Exit Sub-Modules ", "State(s) in (\"\")"=w149, "State(s) at Back (\"\")"="Data: Cleanup\nExit") -> ("States Out"=w148:string)  [unwired: 12 in]
        n49 = call <vilib>:"Add State(s) to Queue__JKI_lib_State_Machine.vi"("State(s) in Front (\"\")"=w148, "State(s) in (\"\")"=w154) -> ("States Out"=w153:string)  [unwired: 13 in]
      }
      frame "---------- API ----------" {
        # "#CSM \"Category Seperator\"\nDo not put any code in this frame."
        n50 = call <vilib>:"Add State(s) to Queue__JKI_lib_State_Machine.vi"("State(s) in (\"\")"=w159) -> ("States Out"=w158:string)  [unwired: 14 in]
      }
      frame "API: Start" {
        # "#CSM API Example\nCopy/Rename this case for your own API"
        n51 = Unbundle By Name(w163) -> ("State"=w168:T4, "Repeat.步骤开始周期"=w161:i32)
        n52 = case shown="\"Idle\"" w168 {
          selector: w168 -> [_ w182 w184]
          tunnel: [Repeating_States."Repeating" ("Acquisition State") w182 w184] -> w169
          tunnel: ["Repeat: Initialize \nRepeat: Judge\nContinuous Check >> Repeat: Judge -><loop> \nRepeat: Stop\nRepeat: Close " ("State(s) in Front (\"\")") _ _] -> w167
          tunnel: [w170 w181 w183] -> w162
          tunnel: w161 -> [_ w181 w183]
          frame "Idle" {
            # "If the system is idle, start the acquisition."
            n53 = call "CSM Get Module Attribute.vim"("CSM Name"="OP1", "Attribute"="当前周期", "Default Value (Empty Variant)"=0 ("Repeat.周期值"), "Wait (5000 ms)"=500 ("Default Value (Empty Variant)")) -> ("Found"=w173:bool, "Value"=w172:i32, "error out"=w174:errorcluster)  [unwired: 7 in, 2 out]
            n54 = call <vilib>:"Clear Errors.vi"("error in (no error)"=w174) -> ()  [unwired: 5 in, 2 out]
            n55 = Select(t=w172, s=w173, f=0) -> (s? t:f=w170:i32)
          }
          frame "Repeating" {
            # "The system is already acquiring. Ignore the \"Start\" message."
          }
          frame "Error" {
          }
        }
        n56 = call <userlib>:"CSMLS - Define Loop State(s).vi"("Loop States"=w167, "States Queue"=w165) -> ("Remaining States"=w164:string)  [unwired: 13 in]
        n57 = Bundle By Name(cluster=w163, "State"=w169, "Repeat.步骤开始周期"=w162) -> (w166:T7)
      }
      frame "API: Stop" {
        # "#CSM API Example\nCopy/Rename this case for your own API"
        n58 = Unbundle By Name(w188) -> ("State"=w189:T4)
        n59 = case shown="\"Repeating\"" w189 {
          tunnel: [_ "Break Continuous" ("State(s) in Front (\"\")") _] -> w185
          frame "Idle" {
            # "The system is already idle. Ignore the \"Stop\" message."
          }
          frame "Repeating" {
            # "If the system is acquiring, stop the acquisition."
          }
          frame "Error" {
          }
        }
        n60 = call <vilib>:"Add State(s) to Queue__JKI_lib_State_Machine.vi"("State(s) in Front (\"\")"=w185, "State(s) in (\"\")"=w187) -> ("States Out"=w186:string)  [unwired: 13 in]
      }
      frame "API: CSM Name" {
        n61 = Bundle By Name(cluster=w192, "CSM Name"=w193) -> (w191:T7)
      }
      frame "API: Steps" {
        n62 = call <vilib>:"Build State String with Arguments__JKI_lib_State_Machine.vi"("Arguments (\"\")"=w196, "State"="Repeat Changed" ("Status with Arguments")) -> ("State with Arguments"=w199:string)  [unwired: 4 in]
        n63 = call <userlib>:"CSM - Broadcast Status Change.vi"("Status With Arguments"=w199, "State Queue"=w198) -> ("Remaining States"=w197:string)  [unwired: 13 in]
      }
      frame "API: INI Read" {
        w205 = T1 [{"行程"=25, "周期"=60, "进度"=1.000390362739563, "光谱测量拿起"=FALSE, "运行方向"=FALSE}, {"行程"=26, "周期"=60, "进度"=1.0013926823933919, "光谱测量拿起"=TRUE, "运行方向"=FALSE}, {"行程"=25, "周期"=60, "进度"=1.0006222248077392, "光谱测量拿起"=FALSE, "运行方向"=FALSE}, {"行程"=26, "周期"=60, "进度"=0.6612281163533529, "光谱测量拿起"=TRUE, "运行方向"=FALSE}]  # 循环步骤
        n64 = call "Convert API String Arguments to Data.vim"("Reference Type"=w205, "API String"=w206) -> ("Data"=w203:T1)  [unwired: 6 in, 1 out]
        n65 = local write "电机步骤"(w203) -> ()
      }
      frame "---------- Repeat ----------" {
        # "#CSM \"Category Seperator\"\nDo not put any code in this frame."
        n66 = call <vilib>:"Add State(s) to Queue__JKI_lib_State_Machine.vi"("State(s) in (\"\")"=w211) -> ("States Out"=w210:string)  [unwired: 14 in]
      }
      frame "Repeat: Initialize" {
        # "#CSM \"Category Seperator\"\nDo not put any code in this frame."
        n67 = Unbundle By Name(w220) -> ("Repeat.步骤开始周期"=w219:i32)
        n68 = disable-structure shown="启用" {
          disable-tunnel: w219 -> [w235 _]
          disable-tunnel: [w229 _] -> w218
          disable-tunnel: [w228 _] -> w215
          frame Enabled {
            n69 = call "CSM Get Module Attribute.vim"("CSM Name"="OP1", "Attribute"="当前周期", "Default Value (Empty Variant)"=0 ("Repeat.周期值"), "Wait (5000 ms)"=500) -> ("Found"=w232:bool, "Value"=w233:i32, "error out"=w231:errorcluster)  [unwired: 7 in, 2 out]
            n70 = call <vilib>:"Clear Errors.vi"("error in (no error)"=w231) -> ()  [unwired: 5 in, 2 out]
            n71 = Select(t=w233, s=w232, f=0) -> (s? t:f=w229:i32)
            n72 = Greater?(x=w229, y=w235) -> (0:w228:bool)
          }
          frame Disabled {
          }
        }
        n73 = Array Size(array="电机步骤") -> (size(s)=w226:i32)
        n74 = for {
          N: w226 -> [_]
          tunnel: [w239] -> w224 mode=indexing
          i -> [w239]
        }
        n75 = Get Date/Time In Seconds() -> (seconds since 1Jan1904=w225:timestamp)
        n76 = Select(t="", s=w215, f="Repeat: Initialize") -> (s? t:f=w212:string)
        n77 = Bundle By Name(cluster=w220, "Repeat.电机步骤开始时间"=w225, "Repeat.电机步骤索引"=w224, "Repeat.下一步？"=TRUE ("下一步？"), "Repeat.步骤开始周期"=w218) -> (w227:T7)
        n78 = call <vilib>:"Add State(s) to Queue__JKI_lib_State_Machine.vi"("State(s) in Front (\"\")"=w212, "State(s) in (\"\")"=w216) -> ("States Out"=w217:string)  [unwired: 13 in]
        "当前次数" <- 1 ("当前次数")
      }
      frame "Repeat: Judge" {
        # "#CSM \"Internal State\"\nThis category is used for holding internal states"
        n79 = Unbundle By Name(w246) -> ("State"=w247:T4)
        n80 = case shown="\"Repeating\"" w247 {
          tunnel: [w249 w261 w296] -> w243
          tunnel: w245 -> [w249 w261 w296]
          tunnel: [w248 w266 w295] -> w244
          tunnel: w246 -> [w248 w270 w295]
          tunnel: [_ w257 _] -> w240
          frame "Idle" {
            # "Ignore \"Acquire\" messages when the acquisition is idle."
          }
          frame "Repeating" {
            # "Acquire more data while in the \"Acquiring\" state."
            n81 = local read "电机步骤"() -> (w268:T1)
            n82 = Unbundle By Name(w270) -> ("Repeat.步骤开始周期"=w283:i32, "Repeat.电机步骤索引"=w265:i32[])
            n83 = Index Array(array=w265, index=0 ("索引")) -> (element=w275:i32)
            n84 = Index Array(array=w268, index=w275) -> (element=w281:T9)
            n85 = Array Size(array=w265) -> (size(s)=w264:i32)
            n86 = Decrement(x=w264) -> (x-1=w263:i32)
            n87 = Unbundle By Name(w281) -> ("周期"=w282:i32)
            n88 = local read "当前次数"() -> (w262:i32)
            n89 = call "CSM Get Module Attribute.vim"("CSM Name"="OP1", "Attribute"="当前周期", "Default Value (Empty Variant)"=0 ("Repeat.周期值"), "Wait (5000 ms)"=500) -> ("Value"=w251:i32, "error out"=w250:errorcluster)  [unwired: 7 in, 3 out]
            n90 = Equal?(x=w275, y=w263) -> (x = y?=w277:bool)
            n91 = Subtract(x=w251, y=w283) -> (x-y=w276:i32)
            n92 = call <vilib>:"Clear Errors.vi"("error in (no error)"=w250) -> ()  [unwired: 5 in, 2 out]
            n93 = Greater Or Equal?(x=w262, y="运行次数") -> (x >= y?=w280:bool)
            n94 = Greater Or Equal?(x=w276, y=w282) -> (x >= y?=w278:bool)
            n95 = Divide(x=w276, y=w282) -> (x/y=w273:dbl)
            n96 = Compound Arithmetic op=AND ("复合运算")(w278, w277) -> (w279:bool)
            n97 = case shown="True" w278 {
              tunnel: w265 -> [w290 w294]
              tunnel: [w290 w293] -> w274
              tunnel: [FALSE TRUE] -> w256
              frame False {
              }
              frame True {
                n98 = Rotate 1D Array(1:w294, 2:-1 ("n")) -> (0:w293:i32[])
              }
            }
            n99 = case shown="True" w279 {
              tunnel: w280 -> [_ w285]
              tunnel: [_ w284] -> w260
              frame False {
              }
              frame True {
                n100 = case shown="False" w285 {
                  tunnel: [_ TRUE] -> w284
                  frame False {
                    n101 = local read "当前次数"() -> (w286:i32)
                    n102 = Increment(x=w286) -> (x+1=w287:i32)
                    n103 = local write "当前次数"(w287) -> ()
                  }
                  frame True {
                  }
                }
              }
            }
            n104 = Bundle By Name(cluster=w281, "进度"=w273) -> (w272:T9)
            n105 = Replace Array Subset(array=w268, new element=w272, index=w275) -> (w267:T1)
            n106 = local write "电机步骤"(w267) -> ()
            n107 = Bundle By Name(cluster=w270, "Repeat.电机步骤索引"=w274, "Repeat.下一步？"=w256) -> (w266:T7)
            n108 = Select(t="Break Continuous", s=w260, f="Repeat: Func") -> (s? t:f=w257:string)
          }
          frame "Error" {
          }
        }
        n109 = call <vilib>:"Add State(s) to Queue__JKI_lib_State_Machine.vi"("State(s) in Front (\"\")"=w240, "State(s) in (\"\")"=w241) -> ("States Out"=w242:string)  [unwired: 13 in]
      }
      frame "Repeat: Func" {
        n110 = Unbundle By Name(w307) -> ("CSM Name"=w302:string, "Repeat.下一步？"=w320:bool, "Repeat.电机步骤索引"=w316:i32[], "Repeat.电机步骤开始时间"=w312:timestamp, "Repeat.步骤开始周期"=w300:i32)
        n111 = local read "电机步骤"() -> (w305:T1)
        n112 = Index Array(array=w316, index=0 ("索引")) -> (element=w317:i32)
        n113 = feedback #1(-1 ("索引")) -> (w311:i32)
        n114 = feedback-in #1(w317) -> ()
        n115 = Index Array(array=w305, index=w317) -> (element=w315:T9)
        n116 = Not Equal?(x=w317, y=w311) -> (x != y?=w319:bool)
        n117 = Unbundle By Name(w315) -> ("光谱测量拿起"=w314:bool, "行程"=w318:i32, "运行方向"=w297:bool)
        n118 = Compound Arithmetic op=OR ("复合运算")(w320, w319) -> (w298:bool)
        n119 = case shown="True" w298 {
          tunnel: w314 -> [_ w323]
          tunnel: w318 -> [_ w325]
          tunnel: w302 -> [_ w327]
          tunnel: ["" ("States Out") w326] -> w301
          tunnel: w297 -> [_ w324]
          frame False {
          }
          frame True {
            n120 = case shown="False" w323 {
              selector: w323 -> [_ w350]
              tunnel: w327 -> [w332 w349]
              tunnel: ["" ("States") w353] -> w326
              tunnel: w325 -> [w330 w352]
              tunnel: w324 -> [w331 w351]
              frame False {
                n121 = Equal To 0?(x=w330) -> (x = 0?=w329:bool)
                n122 = stacked-sequence {
                  tunnel: w332 -> [w335 _]
                  tunnel: w331 -> [w336 _]
                  tunnel: w330 -> [w334 _]
                  tunnel: w329 -> [w333 _]
                  frame #0 {
                    n123 = case shown="False" w333 {
                      tunnel: w334 -> [w345 _]
                      tunnel: w336 -> [w343 _]
                      tunnel: w335 -> [w338 _]
                      frame False {
                        n124 = call "Convert Data To API String Arguments.vim"("Data"=w345) -> ("API String"=w340:string)  [unwired: 7 in, 1 out]
                        n125 = call "Convert Data To API String Arguments.vim"("Data"=w343) -> ("API String"=w339:string)  [unwired: 7 in, 1 out]
                        n126 = call-poly <userlib>:"Build Message with Arguments++.vi"("States With Replace Token"="Action: Change Distance >> <1> -@ <param>\nAction: Direction >> <2> -@ <param>\nAction: RunStart -@ <param>", "<param>"=w338, "<1>"=w340, "<2>"=w339) -> ("States"=w341:string)  [unwired: 11 in]
                        n127 = call <userlib>:"CSM - Run Script.vi"("CSM Scripts"=w341) -> ("error out"=w337:errorcluster)  [unwired: 12 in, 2 out]
                        n128 = call <vilib>:"Clear Errors.vi"("error in (no error)"=w337) -> ()  [unwired: 5 in, 2 out]
                        n129 = Wait (ms)(milliseconds to wait=u32 3000 ("等待时间（毫秒）")) -> ()  [unwired: 1 out]
                      }
                      frame True {
                      }
                    }
                  }
                  frame #1 {
                    n130 = call <userlib>:"CSM - Run Script.vi"("CSM Scripts"="API: Probe Up False -@ OP1") -> ("error out"=w347:errorcluster)  [unwired: 12 in, 2 out]
                    n131 = call <vilib>:"Clear Errors.vi"("error in (no error)"=w347) -> ()  [unwired: 5 in, 2 out]
                  }
                }
              }
              frame True {
                n132 = Equal To 0?(x=w352) -> (x = 0?=w348:bool)
                n133 = stacked-sequence {
                  tunnel: w350 -> [_ _]
                  tunnel: w352 -> [_ w359]
                  tunnel: w351 -> [_ w357]
                  tunnel: [_ w361] -> w353
                  tunnel: w349 -> [_ w360]
                  tunnel: w348 -> [_ w358]
                  frame #0 {
                    n134 = call <userlib>:"CSM - Run Script.vi"("CSM Scripts"="API: Probe Up True -@ OP1") -> ("error out"=w354:errorcluster)  [unwired: 12 in, 2 out]
                    n135 = call <vilib>:"Clear Errors.vi"("error in (no error)"=w354) -> ()  [unwired: 5 in, 2 out]
                    n136 = Wait (ms)(milliseconds to wait=u32 200 ("等待时间（毫秒）")) -> ()  [unwired: 1 out]
                  }
                  frame #1 {
                    n137 = case shown="False" w358 {
                      tunnel: w357 -> [w365 _]
                      tunnel: w359 -> [w364 _]
                      tunnel: w360 -> [w363 _]
                      tunnel: [w362 "" ("States")] -> w361
                      frame False {
                        n138 = call "Convert Data To API String Arguments.vim"("Data"=w364) -> ("API String"=w367:string)  [unwired: 7 in, 1 out]
                        n139 = call "Convert Data To API String Arguments.vim"("Data"=w365) -> ("API String"=w366:string)  [unwired: 7 in, 1 out]
                        n140 = call-poly <userlib>:"Build Message with Arguments++.vi"("States With Replace Token"="Action: Change Distance >> <1> -@ <param>\nAction: Direction >> <2> -@ <param>\nAction: RunStart -@ <param>", "<param>"=w363, "<1>"=w367, "<2>"=w366) -> ("States"=w362:string)  [unwired: 11 in]
                      }
                      frame True {
                      }
                    }
                  }
                }
              }
            }
          }
        }
        n141 = case shown="True" w319 {
          tunnel: [w371 w373] -> w313
          tunnel: w312 -> [w371 _]
          tunnel: w300 -> [w370 _]
          tunnel: [w370 w372] -> w299
          frame False {
          }
          frame True {
            n142 = disable-structure shown="启用" {
              disable-tunnel: [w375 _] -> w372
              frame Enabled {
                n143 = call "CSM Get Module Attribute.vim"("CSM Name"="OP1", "Attribute"="当前周期", "Default Value (Empty Variant)"=0 ("Repeat.周期值")) -> ("Value"=w375:i32, "error out"=w374:errorcluster)  [unwired: 8 in, 3 out]
                n144 = call <vilib>:"Clear Errors.vi"("error in (no error)"=w374) -> ()  [unwired: 5 in, 2 out]
              }
              frame Disabled {
              }
            }
            n145 = Get Date/Time In Seconds() -> (seconds since 1Jan1904=w373:timestamp)
          }
        }
        n146 = Bundle By Name(cluster=w307, "Repeat.下一步？"=FALSE ("下一步？"), "Repeat.电机步骤开始时间"=w313, "Repeat.步骤开始周期"=w299) -> (w306:T7)
        n147 = call <vilib>:"Add State(s) to Queue__JKI_lib_State_Machine.vi"("State(s) in Front (\"\")"=w301, "State(s) in (\"\")"=w303) -> ("States Out"=w304:string)  [unwired: 13 in]
      }
      frame "Repeat: Stop" {
        # "#CSM \"Internal State\"\nThis category is used for holding internal states"
        n148 = call <vilib>:"Add State(s) to Queue__JKI_lib_State_Machine.vi"("State(s) in (\"\")"=w381) -> ("States Out"=w380:string)  [unwired: 14 in]
      }
      frame "Repeat: Close" {
        w382 = Repeating_States."Idle"  # State
        # "#CSM \"Internal State\"\nThis category is used for holding internal states"
        n149 = Bundle By Name(cluster=w384, "State"=w382) -> (w383:T7)
        n150 = call <vilib>:"Add State(s) to Queue__JKI_lib_State_Machine.vi"("State(s) in (\"\")"=w386) -> ("States Out"=w385:string)  [unwired: 14 in]
      }
      frame "---------- Loop ----------" {
        # "#CSM \"Internal State\"\nThis category is used for holding internal states"
        n151 = call <vilib>:"Add State(s) to Queue__JKI_lib_State_Machine.vi"("State(s) in (\"\")"=w389) -> ("States Out"=w388:string)  [unwired: 14 in]
      }
      frame "Continuous Check" {
        # "#CSM \"Internal State\"\nThis category is used for holding internal states"
        n152 = Wait (ms)(milliseconds to wait=u32 75 ("等待时间（毫秒）")) -> ()  [unwired: 1 out]
        n153 = call <userlib>:"CSMLS - Append Continuous State.vi"("Loop State(s) And Arguments"=w391, "Continous Arguments (\"\")"=w391, "Continous State"=w393, "States Queue"=w394) -> ("Remaining States"=w392:string)  [unwired: 7 in]
      }
      frame "Break Continuous" {
        n154 = call <userlib>:"CSMLS - Remove Loop Tag to Break.vi"("States Queue"=w398) -> ("Remaining States"=w396:string)  [unwired: 10 in]
      }
    }
  }
  n155 = while {
    shift-right: [w410] -> _
    shift-left: enum16{"Idle", "Initialize", "Exit"}."Initialize" -> [w411]
    tunnel: "CSM Name" -> [w408]
    shift-right: [w406] -> _
    shift-left: w5 -> [w407]
    shift-right: [w404] -> _
    shift-left: -1 -> [w405]
    shift-right: [w403] -> _
    shift-left: _ -> [w402]
    shift-right: [w401] -> _
    shift-left: _ -> [w400]
    stop <- w409 stop-if-true
    n156 = case shown="\"Idle\", 默认" w411 {
      tunnel: [enum16{"Idle", "Initialize", "Exit"}."Idle" w429 enum16{"Idle", "Initialize", "Exit"}."Exit"] -> w410
      tunnel: [_ _ TRUE] -> w409
      tunnel: w408 -> [w415 w428 _]
      tunnel: w407 -> [w418 w426 w456]
      tunnel: [w418 w427 w456] -> w406
      tunnel: w405 -> [_ w424 _]
      tunnel: [-1 w425 _] -> w404
      tunnel: [w414 w422 _] -> w403
      tunnel: w402 -> [_ w423 w455]
      tunnel: [w412 w420 w453] -> w401
      tunnel: w400 -> [_ w421 w453]
      frame "Initialize" {
        w413 = FALSE  # your data
        n157 = call <userlib>:"CSM - Module Exit Event.vi"("Name (\"\" to Use UUID) In"=w415) -> ("CSM Exit Event"=w416:refnum<user-event>)  [unwired: 8 in, 2 out]
        n158 = register-events(w416) -> (reference out=w414:refnum<event-registration>)  [unwired: 2 in, 1 out]
        n159 = Bundle("your data"=w413) -> (w412:cluster{"your data":bool})  [unwired: 1 in]
      }
      frame "Idle", Default {
        n160 = event shown="[3] \"电机步骤\": 值改变" {
          selector: w423 -> [_ _ _ _]
          dyn-events: [_ _ _ _] -> w422
          timeout: w424 -> [_ _ _ _]
          tunnel: [_ enum16{"Idle", "Initialize", "Exit"}."Exit" _ _] -> w429
          tunnel: w428 -> [w431 _ _ _]
          tunnel: w426 -> [w434 w438 w443 w450]
          tunnel: [w432 w438 w444 w451] -> w427
          tunnel: [-1 _ _ _] -> w425
          tunnel: w421 -> [w430 w436 w445 w452]
          tunnel: [w430 w436 w445 w452] -> w420
          event Timeout {
            n161 = event-data() -> ()  [unwired: 1 in, 3 out]
            n162 = call-poly <userlib>:"CSM - Filter JKISM String Queue.vi"("States In"=w434) -> ("States Out"=w433:string)  [unwired: 14 in]
            n163 = call <userlib>:"CSM - Forward UI Operations to CSM.vi"("Name (\"\" to Use UUID)"=w431, "State(s) In (\"\")"=w433) -> ("States Out"=w432:string)  [unwired: 8 in, 1 out]
          }
          event User Event {
            n164 = event-data() -> ()  [unwired: 1 in, 1 out]
          }
          event "循环开始": Value Change {
            n165 = event-data() -> ()  [unwired: 1 in, 1 out]
            n166 = Select(t="API: Start", s="循环开始", f="API: Stop") -> (s? t:f=w439:string)
            n167 = call <vilib>:"Add State(s) to Queue__JKI_lib_State_Machine.vi"("State(s) in Front (\"\")"=w439, "State(s) in (\"\")"=w443) -> ("States Out"=w444:string)  [unwired: 13 in]
          }
          event Value Change {
            n168 = event-data() -> ("NewVal"=w449:T1)  [unwired: 1 in]
            n169 = call "Convert Data To API String Arguments.vim"("Data"=w449) -> ("API String"=w448:string)  [unwired: 7 in, 1 out]
            n170 = call <vilib>:"Build State String with Arguments__JKI_lib_State_Machine.vi"("Arguments (\"\")"=w448, "State"="API: Steps") -> ("State with Arguments"=w446:string)  [unwired: 4 in]
            n171 = call <vilib>:"Add State(s) to Queue__JKI_lib_State_Machine.vi"("State(s) in Front (\"\")"=w446, "State(s) in (\"\")"=w450) -> ("States Out"=w451:string)  [unwired: 13 in]
          }
        }
      }
      frame "Exit" {
        n172 = Unregister For Events(event registration refnum=w455) -> (error out=w454:errorcluster)  [unwired: 1 in]
        n173 = call <vilib>:"Clear Errors.vi"("error in (no error)"=w454) -> ()  [unwired: 5 in, 2 out]
      }
    }
  }
  n174 = call <userlib>:"CSM - Sync Configuration Variables to File.vi"("All Temp Variable to Default Ini(F)"=TRUE, "error in (no error)"=w2) -> ()  [unwired: 7 in, 1 out]
